vi "Lab02_task3.vi"() -> ()   [LabVIEW 2022 SP3]
uses:
  <vilib>/Analysis/1siggen.llb/Ramp Pattern by Samples.vi
  <vilib>/Utility/file.llb/Write Delimited Spreadsheet (DBL).vi
  <vilib>/Analysis/NI_AALBase.lvlib
panel:
  in  "file path (dialog if empty)":path
  out "XY Graph":cluster{"Ramp Pattern":dbl[], dbl[]}(graph)
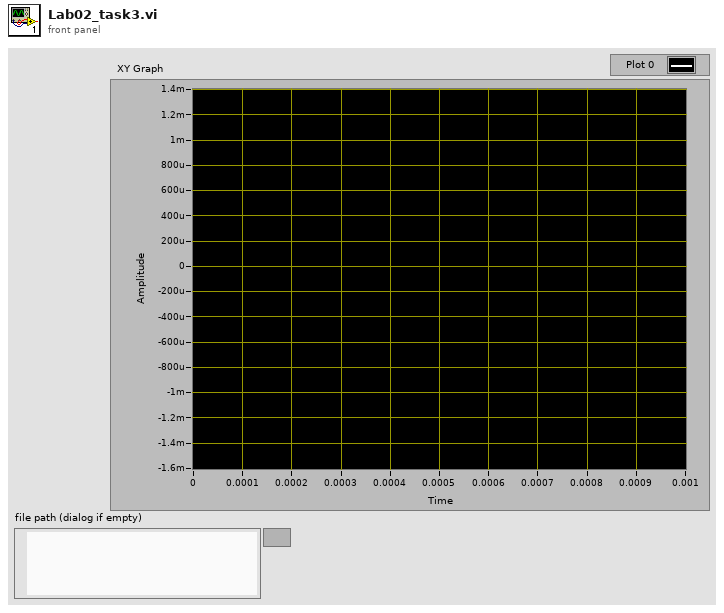
[diagram p1: front panel]
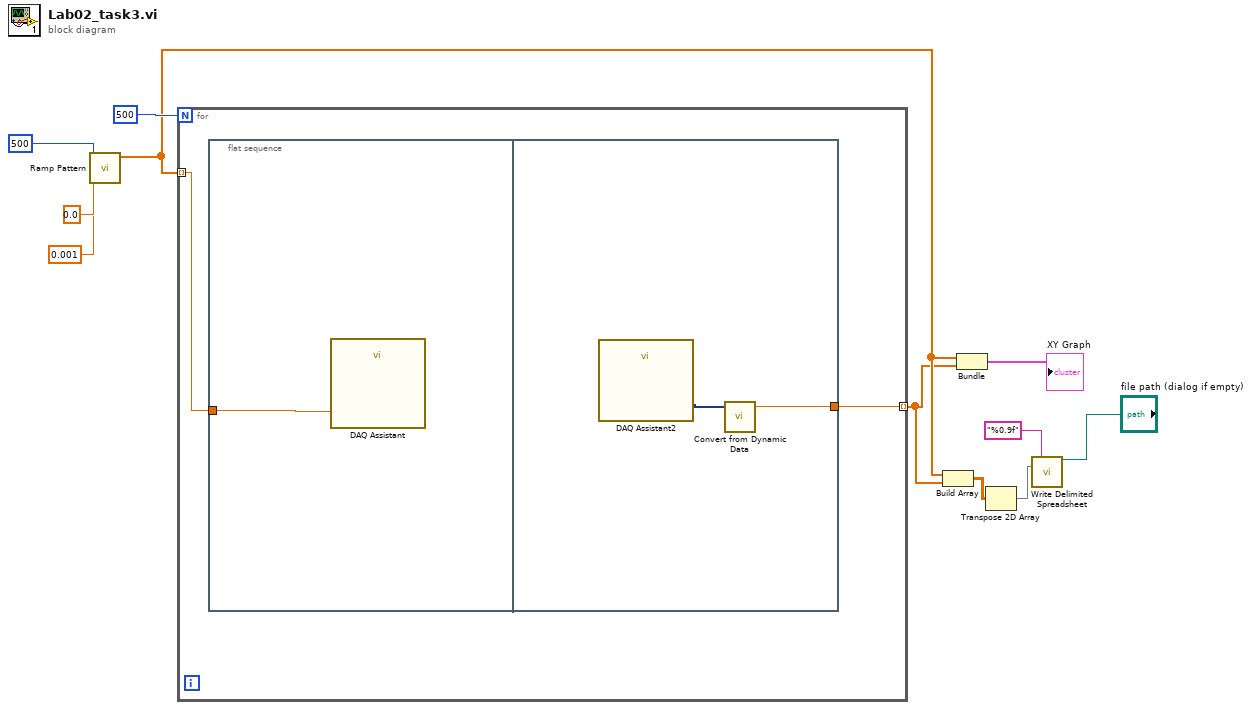
[diagram p0: block diagram]
diagram:
  n1 = call-poly <vilib>:"Ramp Pattern.vi"("start"=0.0, "end"=0.001, "samples"=500) -> ("Ramp Pattern"=w3:dbl[])  [unwired: 7 in, 1 out]
  n2 = for {
    N: 500 -> [_]
    tunnel: w3 -> [w13] mode=indexing
    tunnel: [w12] -> w2 mode=indexing
    n3 = flat-sequence {
      tunnel: w13 -> [w14]
      tunnel: [w15] -> w12
      frame #0 {
        n4 = call "DAQ Assistant"("data"=w14) -> ()  [unwired: 17 in, 2 out]
      }
      frame #1 {
        n5 = call "DAQ Assistant2"() -> ("data"=w16:dynamicdata)  [unwired: 17 in, 2 out]
        n6 = call "Convert from Dynamic Data"("Dynamic Data Type"=w16) -> ("Scalar"=w15:dbl)  [unwired: 3 in]
      }
    }
  }
  n7 = Build Array(w3, w2) -> (w6:dbl[][])
  n8 = Bundle("Ramp Pattern"=w3, w2) -> (→"XY Graph":cluster{"Ramp Pattern":dbl[], dbl[]})  [unwired: 1 in]
  n9 = Transpose 2D Array(2D array=w6) -> (transposed array=w5:dbl[][])
  n10 = call-poly <vilib>:"Write Delimited Spreadsheet.vi"("file path (dialog if empty)"="file path (dialog if empty)", "format (%.3f)"="%0.9f", "2D data"=w5) -> ()  [unwired: 11 in, 2 out]
